vi "Benchmark mupExpr_parse_and_eval.vi"(8 "error in (no error)":errorcluster, 10 "Iterations":i32=10000, 11 "Expression":string="5*x^2+2*x+20") -> (0 "error out":errorcluster, 2 "x":dbl[](array[numeric]), 3 "y":dbl[](array[numeric]), 5 "dt average":dbl)   [LabVIEW 2015]
uses:
  mupExpr/mupExpr.lvclass
  mupExpr/mupExpr.lvclass/mupExpr.ctl
  mupLib/mupEval.vi
  mupLib/mupSetVarValue.vi
  mupLib/mupCheckError.vi
  <vilib>/Utility/error.llb/Error Cluster From Error Code.vi
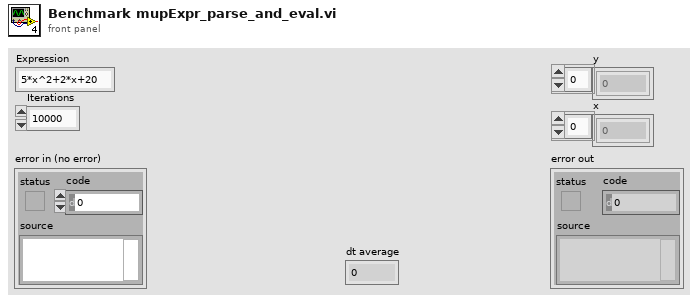
[diagram p1: front panel]
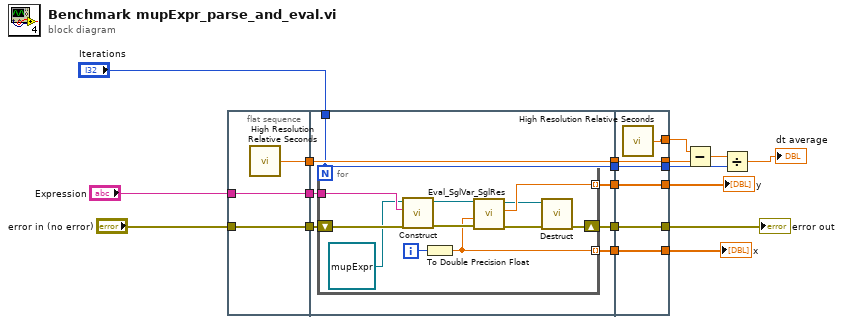
[diagram p0: block diagram]
diagram:
  n1 = flat-sequence {
    tunnel: "error in (no error)" -> [w22]
    tunnel: [w22] -> w17
    tunnel: [w21] -> w12
    tunnel: [w20] -> w4
    tunnel: "Expression" -> [w20]
    tunnel: w17 -> [w29]
    tunnel: [w28] -> w16
    tunnel: [w27] -> w15
    tunnel: [w26] -> w14
    tunnel: [w25] -> w13
    tunnel: w12 -> [w25]
    tunnel: "Iterations" -> [w24]
    tunnel: [w24] -> w6
    tunnel: w4 -> [w23]
    tunnel: [w44] -> w18
    tunnel: [w45] -> w19
    tunnel: [w46] -> w1
    tunnel: w16 -> [w46]
    tunnel: w15 -> [w45]
    tunnel: w14 -> [w44]
    tunnel: [w43] -> w10
    tunnel: w13 -> [w43]
    tunnel: [w42] -> w11
    tunnel: [w41] -> w7
    tunnel: w6 -> [w41]
    frame #0 {
      n2 = call <vilib>:"High Resolution Relative Seconds.vi"() -> ("relative seconds"=w21:dbl)
    }
    frame #1 {
      n3 = for {
        N: w24 -> [_]
        shift-right: [w32] -> w28
        shift-left: w29 -> [w35]
        tunnel: [w39] -> w27 mode=indexing
        tunnel: [w31] -> w26 mode=indexing
        tunnel: w23 -> [w38]
        i -> [w40]
        n4 = call-dynamic "Construct.vi"("error in (no error)"=w35, "Expression"=w38, "muExpr in"=refnum<class "mupExpr.lvclass"> refnum) -> ("error out"=w36:errorcluster, "mupExpr out"=w37:refnum<class "mupExpr.lvclass">)  [unwired: 5 in, 2 out]
        n5 = To Double Precision Float(number=w40) -> (double precision float=w31:dbl)
        n6 = call "Eval_SglVar_SglRes.vi"("error in (no error)"=w36, "varValue"=w31, "muExpr in"=w37) -> ("error out"=w34:errorcluster, "Result"=w39:dbl, "muExpr out"=w33:refnum<class "mupExpr.lvclass">)  [unwired: 6 in]
        n7 = call-dynamic "Destruct.vi"("error in (no error)"=w34, "muExpr in"=w33) -> ("error out"=w32:errorcluster)  [unwired: 9 in]
      }
    }
    frame #2 {
      n8 = call <vilib>:"High Resolution Relative Seconds.vi"() -> ("relative seconds"=w42:dbl)
    }
  }
  n9 = Subtract(x=w11, y=w10) -> (x-y=w8:dbl)
  n10 = Divide(x=w8, y=w7) -> (x/y=→"dt average":dbl)
  "y" <- w19
  "x" <- w18
  "error out" <- w1
